vi "Neopixel_Control_Individual_Ex.vi"() -> ()   [LabVIEW 2026]
panel:
  in  "Num_Neo":u8
  out "error out":errorcluster
  in  "Stop Button":bool
  out "respuesta":string
  in  "Color Box":u32(colorbox)
  in  "VISA resource name":refnum<visa-resource-name>
  in  "Opcion":u8
  # "Ejemplo: Neopixel Control Individual"
  # "Descripción: enciende el pixel individual del color seleccionado"
  # "Configuracion"
  # "Indicadores"
  # "Control"
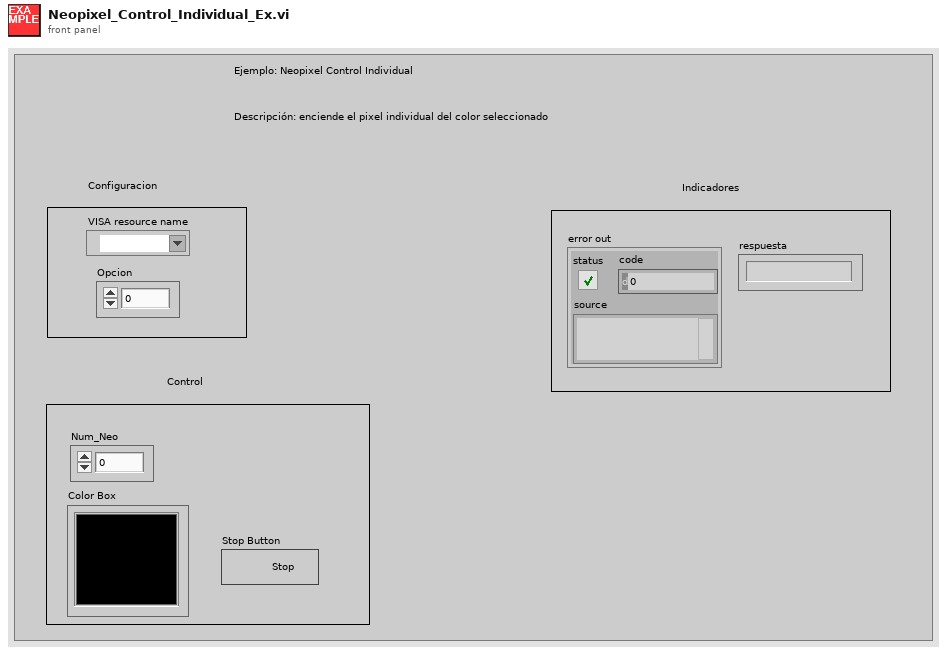
[diagram p1: front panel]
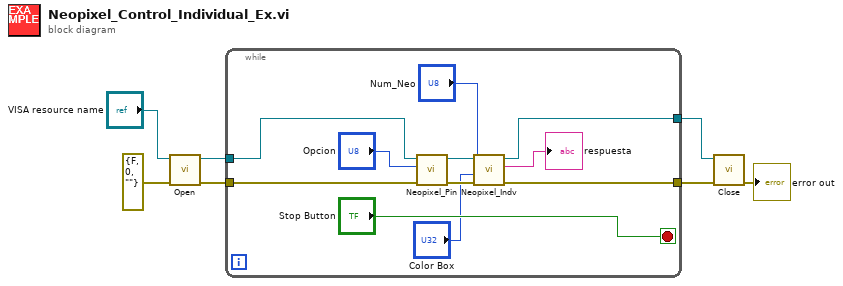
[diagram p0: block diagram]
diagram:
  n1 = call "Open.vi"("error in (no error)"=errorcluster {"status"=FALSE, "code"=0, "source"=""}, "VISA resource name"="VISA resource name") -> ("error out"=w6:errorcluster, "VISA resource name out"=w7:refnum<visa-resource-name>)  [unwired: 8 in]
  n2 = while {
    tunnel: w7 -> [w18]
    tunnel: [w14] -> w3
    tunnel: w6 -> [w17]
    tunnel: [w13] -> w2
    stop <- "Stop Button" stop-if-true
    n3 = call "Neopixel_Pin.vi"("error in (no error)"=w17, "Opcion"="Opcion", "VISA resource name"=w18) -> ("error out"=w12:errorcluster, "VISA resource name out"=w15:refnum<visa-resource-name>)  [unwired: 6 in, 1 out]
    n4 = call "Neopixel_Indv.vi"("VISA resource name"=w15, "Num_Neo"="Num_Neo", "Color Box"="Color Box", "error in (no error)"=w12) -> ("VISA resource name out"=w14:refnum<visa-resource-name>, "respuesta"=→"respuesta":string, "error out"=w13:errorcluster)  [unwired: 4 in]
  }
  n5 = call "Close.vi"("error in (no error)"=w2, "VISA resource name"=w3) -> ("error out"=→"error out":errorcluster)  [unwired: 9 in]
